vi "New Run Trigger.vi"(8 "error in":errorcluster, 11 "CaptureDetectionLoopDataIn":T1={"Period"=-1, "Reset"=TRUE, "Iteration"=0, "Capture"=path "", "Mode"={"Replay"=enum."None", "Record"=enum."None"}, "Replay Run ID"="", "Frame Number"=0, "Core Module ID"=0, "EventRecorderLaunched"=FALSE, "Frame 0 relative seconds"=0.0, "Record Run ID"=""} {"Frame 0 relative seconds" format="%_19f"}) -> (0 "error out":errorcluster, 2 "Latest Frame":path, 3 "CaptureDetectionLoopDataOut":T1={"Period"=-1, "Reset"=TRUE, "Iteration"=0, "Capture"=path "", "Mode"={"Replay"=enum."None", "Record"=enum."None"}, "Replay Run ID"="", "Frame Number"=0, "Core Module ID"=0, "EventRecorderLaunched"=FALSE, "Frame 0 relative seconds"=0.0, "Record Run ID"=""} {"Frame 0 relative seconds" format="%_19f"})   [LabVIEW 2026, in "Launcher.lvlib"]
uses:
  Launcher.lvlib
  Capture detection loop data--cluster.ctl
  Mode.ctl
  ReplayMode.ctl
  RecordMode.ctl
  Core/global.vi
  Core/Core.lvlib
panel:
  out "Record Run ID":string
  out "Numeric":i32
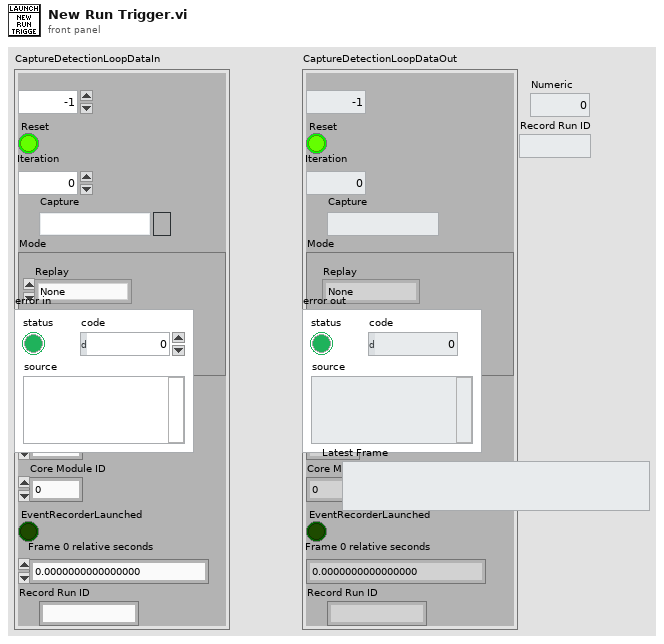
[diagram p1: front panel]
types:
  T1 = typedef "Capture detection loop data--cluster.ctl" = cluster{"Period":i32, "Reset":bool, "Iteration":i32, "Capture":path, "Mode":T2, "Replay Run ID":string, "Frame Number":u32, "Core Module ID":i32, "EventRecorderLaunched":bool, "Frame 0 relative seconds":dbl, "Record Run ID":string}
  T2 = typedef "Mode.ctl" = cluster{"Replay":T3, "Record":T4}
  T3 = typedef "ReplayMode.ctl" = enum16{"None", "User Events"}
  T4 = typedef "RecordMode.ctl" = enum16{"None", "User Events", "Benchmarks", "User Events and Benchmarks"}
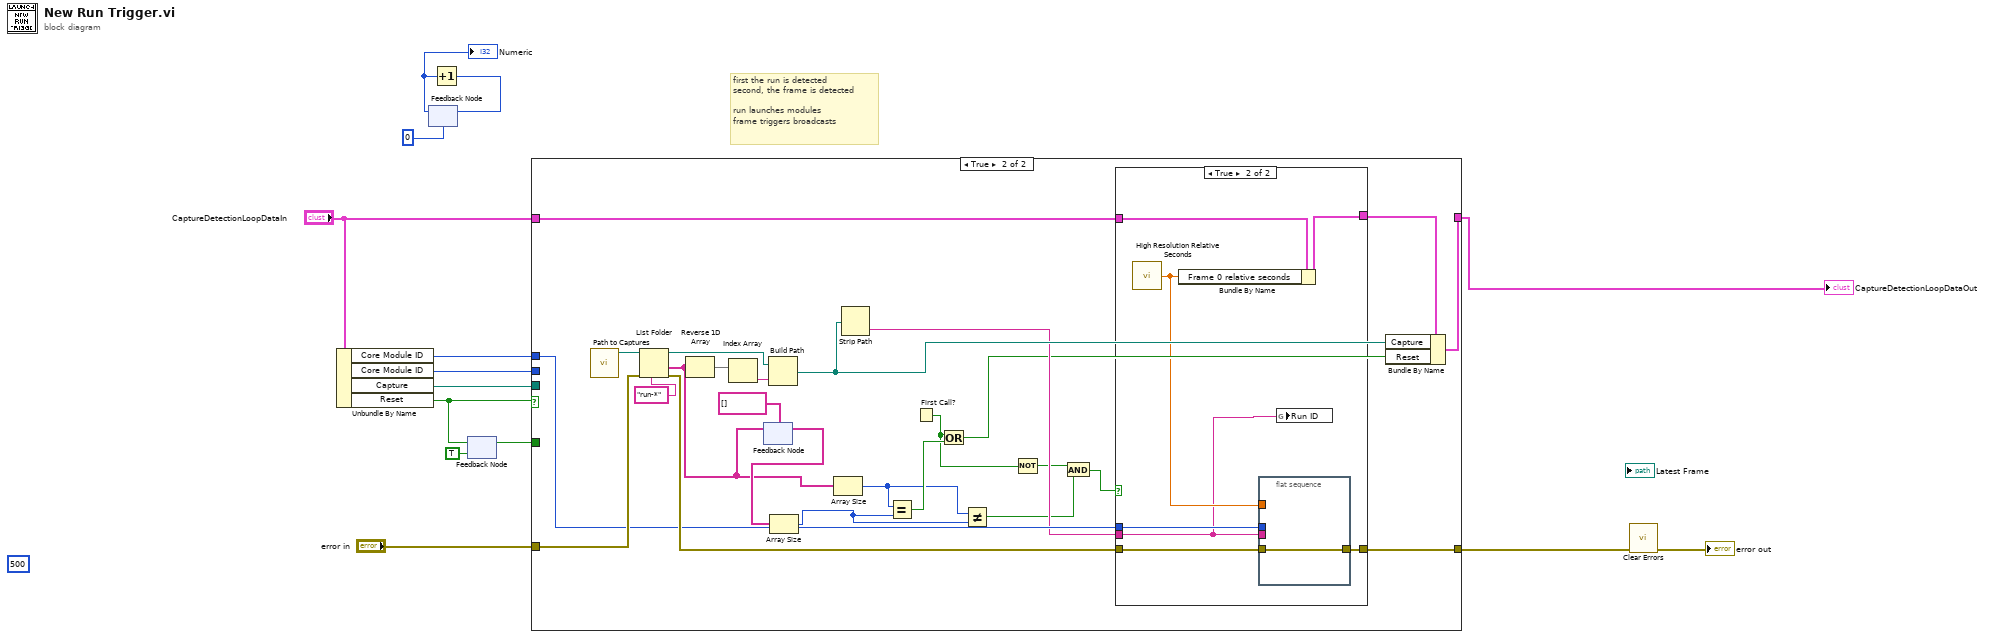
[diagram p0: block diagram]
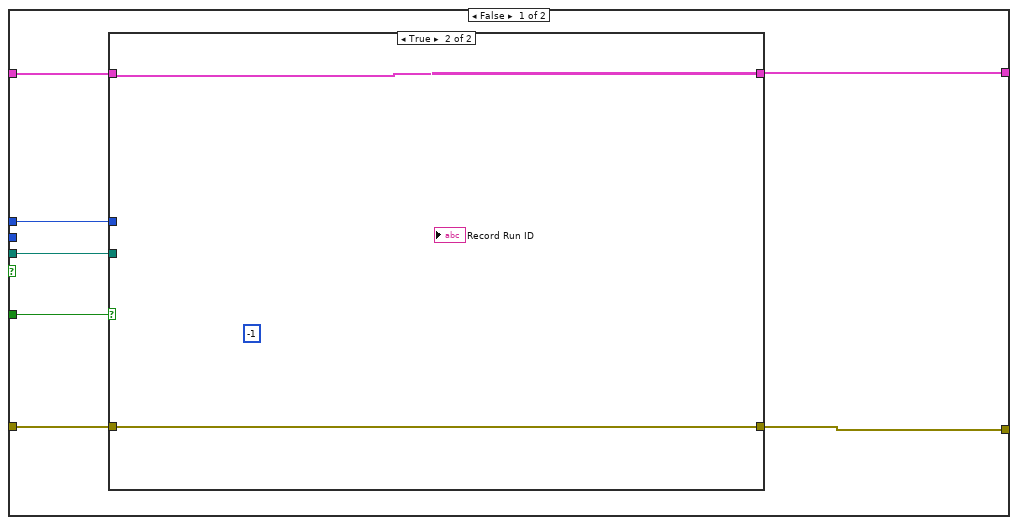
[diagram p2: hidden frame]
diagram:
  (unwired) 500
  # "first the run is detected\nsecond, the frame is detected\n\nrun launches modules\nframe triggers broadcasts"
  n1 = Unbundle By Name("CaptureDetectionLoopDataIn") -> ("Core Module ID"=w2:i32, "Core Module ID"=w3:i32, "Capture"=w12:path, "Reset"=w11:bool)
  n2 = feedback #1(0) -> (w6:i32)
  "Numeric" <- w6
  n3 = Increment(x=w6) -> (x+1=w7:i32)
  n4 = feedback-in #1(w7) -> ()
  n5 = feedback-in #2(w11) -> ()
  n6 = feedback #2(TRUE ("Reset")) -> (w10:bool)
  n7 = case shown="True" w11 {
    tunnel: "error in" -> [w21 w43]
    tunnel: [w20 w37] -> w5
    tunnel: w12 -> [w16 _]
    tunnel: "CaptureDetectionLoopDataIn" -> [w19 w27]
    tunnel: [w18 w50] -> w4
    tunnel: w10 -> [w17 _]
    tunnel: w3 -> [_ _]
    tunnel: w2 -> [w15 w36]
    frame False {
      n8 = case shown="True" w17 {
        tunnel: w21 -> [w23 w25]
        tunnel: [w23 w25] -> w20
        tunnel: w19 -> [w22 w24]
        tunnel: [w22 w24] -> w18
        tunnel: w16 -> [_ _]
        tunnel: w15 -> [_ _]
        frame False {
        }
        frame True {
          (unwired) -1 ("Module ID")
        }
      }
    }
    frame True {
      n9 = call "Path to Captures.vi"() -> ("Captures"=w48:path)  [unwired: 11 in]
      n10 = List Folder(path=w48, pattern="run-*", error in=w43) -> (path out=w47:path, folder names=w41:string[], error out=w38:errorcluster)  [unwired: 1 in, 1 out]
      n11 = Reverse 1D Array(array=w41) -> (reversed array=w45:string[])
      n12 = Index Array(array=w45) -> (element=w46:string)  [unwired: 1 in]
      n13 = feedback-in #3(w41) -> ()
      n14 = feedback #3(string[] [] ("folder names")) -> (w42:string[])
      n15 = Build Path(base path=w47, name or relative path=w46) -> (appended path=w49:path)
      n16 = Array Size(array=w42) -> (size(s)=w32:i32)
      n17 = Array Size(array=w41) -> (size(s)=w33:i32)
      n18 = Strip Path(path=w49) -> (name=w35:string)  [unwired: 1 out]
      n19 = Equal?(x=w33, y=w32) -> (x = y?=w39:bool)
      n20 = First Call?() -> (First Call?: T/F=w31:bool)
      n21 = Or(x=w31, y=w39) -> (x .or. y?=w34:bool)
      n22 = Not Equal?(x=w33, y=w32) -> (x != y?=w29:bool)
      n23 = Not(x=w31) -> (.not. x?=w30:bool)
      n24 = And(x=w30, y=w29) -> (x .and. y?=w28:bool)
      n25 = case shown="True" w28 {
        tunnel: w38 -> [w52 w59]
        tunnel: [w52 w58] -> w37
        tunnel: w36 -> [_ w57]
        tunnel: w35 -> [_ w53]
        tunnel: w27 -> [w51 w56]
        tunnel: [w51 w55] -> w26
        frame False {
        }
        frame True {
          n26 = call <vilib>:"High Resolution Relative Seconds.vi"() -> ("relative seconds"=w54:dbl)
          n27 = Bundle By Name(cluster=w56, "Frame 0 relative seconds"=w54) -> (w55:T1)
          n28 = flat-sequence {
            tunnel: w59 -> [w60]
            tunnel: [w60] -> w58
            tunnel: w57 -> [_]
            tunnel: w53 -> [_]
            tunnel: w54 -> [_]
            frame #0 {
            }
          }
          n29 = global write "global.vi" "Run ID"(w53) -> ()
        }
      }
      n30 = Bundle By Name(cluster=w26, "Capture"=w49, "Reset"=w34) -> (w50:T1)
    }
  }
  "CaptureDetectionLoopDataOut" <- w4
  n31 = call <vilib>:"Clear Errors.vi"("error in (no error)"=w5) -> ("error out"=→"error out":errorcluster)  [unwired: 5 in, 1 out]
